vi "TEST - Array Size(s).vi"(8 "error in (no error)":errorcluster) -> (0 "error out":errorcluster, 2 "pass":bool)   [LabVIEW 2020, in "test_openg_array.lvlib"]
uses:
  test_openg_array.lvlib
  <userlib>/_OpenG.lib/error/error.llb/openg_error.lvlib
  source/library/openg_variant.lvlib
panel:
  out "Failures":T1(array[cluster])
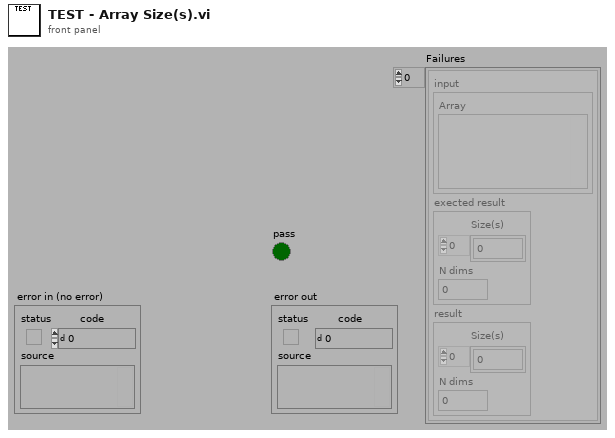
[diagram p1: front panel]
types:
  T1 = cluster{"input":cluster{"Array":variant}, "exected result":cluster{"Size(s)":u32[], "N dims":u32}, "result":cluster{"Size(s)":u32[], "N dims":u32}}[]
  T2 = cluster{"input":cluster{"Array":variant}, "exected result":cluster{"Size(s)":u32[], "N dims":u32}, "result":cluster{"Size(s)":u32[], "N dims":u32}}
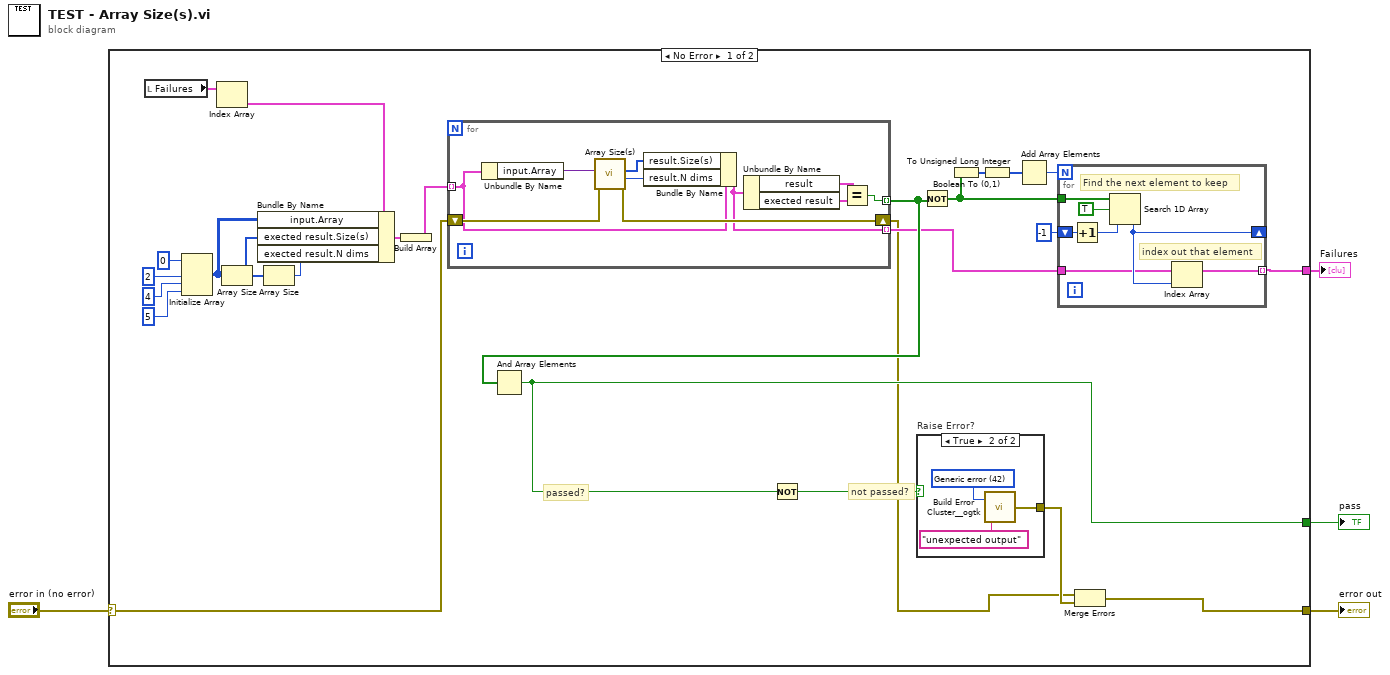
[diagram p0: block diagram]
diagram:
  n1 = case shown="No Error" "error in (no error)" {
    selector: "error in (no error)" -> [w15 w50]
    tunnel: [w26 _] -> w4
    tunnel: [w29 w50] -> w2
    tunnel: [w18 _] -> w1
    frame No Error {
      # "not passed?"
      # "passed?"
      n2 = local read "Failures"() -> (w13:T1)
      n3 = Initialize Array(0, u32 2 ("Numeric"), 4 ("Numeric"), 5 ("Numeric")) -> (w5:i32[][][])
      n4 = Index Array(array=w13) -> (element=w12:T2)  [unwired: 1 in]
      n5 = Array Size(array=w5) -> (size(s)=w7:i32[])
      n6 = Array Size(array=w7) -> (size(s)=w6:i32)
      n7 = Bundle By Name(cluster=w12, "input.Array"=w5, "exected result.Size(s)"=w7, "exected result.N dims"=w6) -> (w17:T2)
      n8 = Build Array(w17) -> (w16:T1)
      n9 = for {
        tunnel: w16 -> [w43] mode=indexing
        tunnel: [w46] -> w20 mode=indexing
        tunnel: [w42] -> w19 mode=indexing
        shift-right: [w44] -> w14
        shift-left: w15 -> [w45]
        n10 = Unbundle By Name(w43) -> ("input.Array"=w37:variant)
        n11 = call "Array Size(s).vi"("error in (no error)"=w45, "Array"=w37) -> ("error out"=w44:errorcluster, "N dims"=w39:u32, "Size(s)"=w40:u32[])  [unwired: 7 in]
        n12 = Bundle By Name(cluster=w43, "result.Size(s)"=w40, "result.N dims"=w39) -> (w42:T2)
        n13 = Unbundle By Name(w42) -> ("result"=w41:cluster{"Size(s)":u32[], "N dims":u32}, "exected result"=w38:cluster{"Size(s)":u32[], "N dims":u32})
        n14 = Equal?(x=w41, y=w38) -> (x = y?=w46:bool)
      }
      n15 = And Array Elements(Boolean array=w20) -> (logical AND=w26:bool)
      n16 = Not(x=w26) -> (.not. x?=w27:bool)
      n17 = case "Raise Error?" shown="True" w27 {
        tunnel: [_ w47] -> w28
        frame False {
        }
        frame True {
          w48 = 42 items=["No error", "Argument error", "Memory is full", "Out of zone", "End of file", "File already open", "Generic file I/O error", "File not found", "File permission error", "Disk is full", "Duplicate path", "Too many files open", "System feature not enabled", "Resource file not found", "Cannot add resource", "Resource not found", "Image not found", "Image memory error", "Pen does not exist", "Config type invalid", "Config token not found", "Config parse error", "Config memory error", "Bad external code format", "Bad external code offset", "External code not present", "Null window", "Destroy window error", "Null menu", "Print aborted", "Bad print record", "Print driver error", "Windows error during printing", "Memory error during printing", "Print dialog error", "Generic print error", "Invalid device refnum", "Device not found", "Device parameter error", "Device unit error", "Cannot open device", "Device call aborted", "Generic error", "Cancelled by user", "Object ID too low", "Object ID too high", "Object not in heap", "Unknown heap", "Unknown object (invalid DefProc)", "Unknown object (DefProc not in table)", "Message out of range", "Invalid (null) method", "Unknown message", "Manager call not supported", "Bad address", "Network operation in progress", "Network operation timed out", "Connection is busy", "Network attribute not supported", "Network error", "Address in use", "System out of memory", "Connection aborted", "Connection refused", "Not connected", "Already connected", "Connection closed", "Initialization error (interapplication manager)", "Bad occurrence", "Wait on unbound occurrence handler", "Occurrence queue overflow", "Datalog type conflict", "Unused", "Unrecognized type (interapplication manager)", "Memory corrupt", "Failed to make temporary DLL", "Old CIN version", "Drag socket not found", "Failed to load drop-object", "Failed to register OLE object", "Failed to release OLE object", "Format specifier type mismatch", "Unknown format specifier", "Too few format specifiers", "Too many format specifiers", "Scan failed", "Newer CIN version", "Error converting to variant", "Runtime menu error", "Password tampered", "Variant attribute not found", "Incompatible variant data type", "Event data is not available", "Event Store is not present", "Occurrence is not found", "Event Queue is not created", "Event info is not available", "Refnum passed is NULL", "Error retrieving Class GUID", "Error retrieving CoClass GUID", "Error retrieving TypeLib GUID.", "Bad built application magic bytes.", "Specific driver is different from the specific driver associated with the Logical Name.", "There is no session opened to the class driver.", "Max Error", "MAX - Error with config objects", "MAX - Error loading configuration", "MAX - Group not supported"]
          n18 = call <userlib>:"Build Error Cluster__ogtk.vi"("String to Prepend to source (\"\")"="unexpected output" ("String to Prepend to source (\"\")"), "code"=w48) -> ("error out"=w47:errorcluster)
        }
      }
      n19 = Not(x=w20) -> (.not. x?=w22:bool[])
      n20 = Boolean To (0,1)(Boolean=w22) -> (0, 1=w23:i16[])
      n21 = To Unsigned Long Integer(number=w23) -> (unsigned 32bit integer=w21:u32[])
      n22 = Add Array Elements(numeric array=w21) -> (sum=w24:u32)
      n23 = for {
        N: w24 -> [_]
        tunnel: w19 -> [w32]
        tunnel: w22 -> [w36]
        shift-right: [w33] -> _
        shift-left: -1 ("start index (0)") -> [w34]
        tunnel: [w31] -> w18 mode=indexing
        # "index out that element"
        # "Find the next element to keep"
        n24 = Increment(x=w34) -> (x+1=w30:i32)
        n25 = Search 1D Array(1D array=w36, element=TRUE, start index (0)=w30) -> (index of element=w33:i32)
        n26 = Index Array(array=w32, index=w33) -> (element=w31:T2)
      }
      n27 = Merge Errors(w14, w28) -> (w29:errorcluster)
    }
    frame Error {
    }
  }
  "pass" <- w4
  "error out" <- w2
  "Failures" <- w1
